vi "Device_Status.vi"(8 "error in (no error)":errorcluster, 11 "CANsub_Channel in":refnum<class "CANsub_Channel.lvclass">) -> (0 "error out":errorcluster, 2 "device status":T1, 3 "CANsub_Channel out":refnum<class "CANsub_Channel.lvclass">)   [LabVIEW 2021, in "CANsub_API.lvlib" / "CANsub_Channel.lvclass"]
doc: "Reads the CAN controller state and the error counters from the device with one REST call. It does not use the WebSocket connection, and it works when the channel is open or closed. Setup/teardown only: do not call in a periodic loop (allocates, may block)."
uses:
  CANsub_Channel.lvclass
  common/Typedefs/CANsub_Device_Status.ctl
  common/CANsub_Common.lvlib
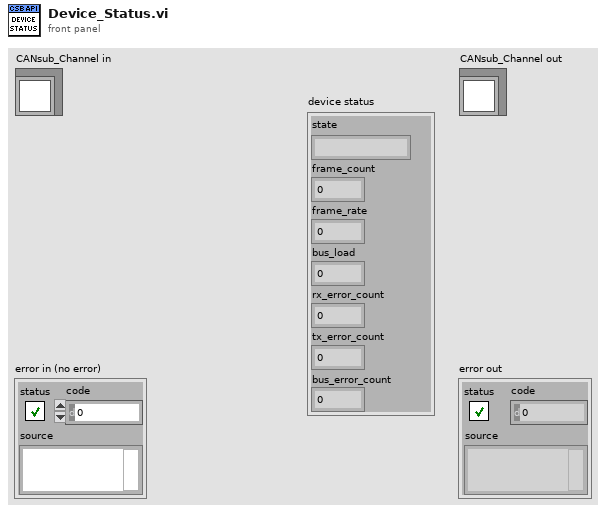
[diagram p1: front panel]
types:
  T1 = typedef "CANsub_Common.lvlib/CANsub_Device_Status.ctl" = cluster{"state":string, "frame_count":u32, "frame_rate":dbl, "bus_load":dbl, "rx_error_count":u32, "tx_error_count":u32, "bus_error_count":u32}
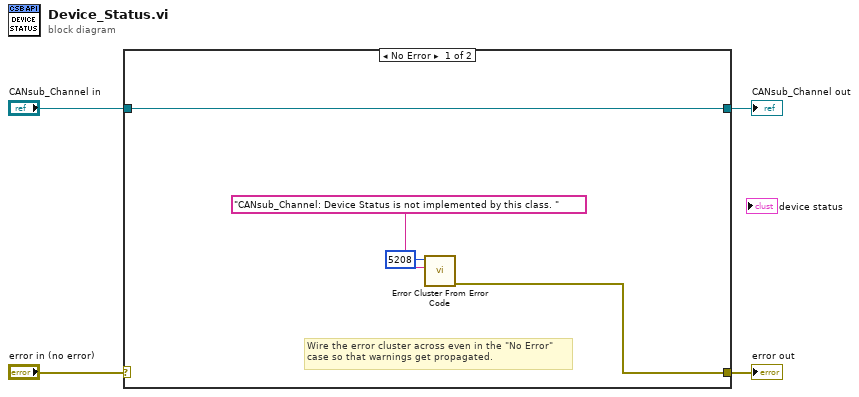
[diagram p0: block diagram]
diagram:
  n1 = case shown="No Error" "error in (no error)" {
    selector: "error in (no error)" -> [_ w10]
    tunnel: [w7 w10] -> w3
    tunnel: [w8 w9] -> w1
    tunnel: "CANsub_Channel in" -> [w8 w9]
    frame No Error {
      # "Wire the error cluster across even in the \"No Error\"\ncase so that warnings get propagated."
      n2 = call <vilib>:"Error Cluster From Error Code.vi"("error message (\"\")"="CANsub_Channel: Device Status is not implemented by this class. " ("error message (\"\")"), "error code (0)"=5208) -> ("error out"=w7:errorcluster)  [unwired: 7 in]
    }
    frame Error {
    }
  }
  "error out" <- w3
  "CANsub_Channel out" <- w1
